vi "Destroy CIF Publisher.vi"(8 "error in (no error)":errorcluster, 11 "Publisher Reference":T1) -> (0 "error out":errorcluster)   [LabVIEW 2021, in "Iceoryx.lvlib"]
uses:
  Iceoryx.lvlib
  SubVIs/Convert Error Core.vi
  Refnum/Typedef/CIF Publisher Refnum.ctl
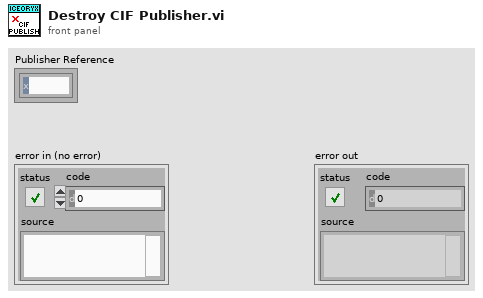
[diagram p1: front panel]
types:
  T1 = typedef "Iceoryx.lvlib/CIF Publisher Refnum.ctl" = refnum<k1>
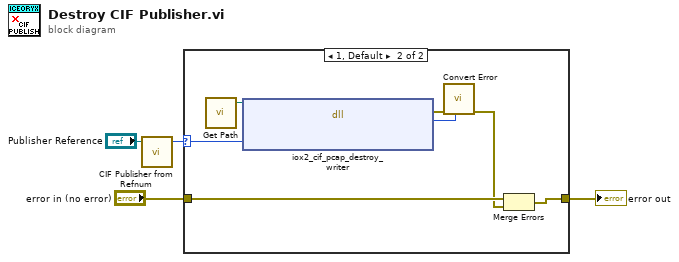
[diagram p0: block diagram]
diagram:
  n1 = call "CIF Publisher from Refnum.vi"("CIF Publisher Refnum"="Publisher Reference") -> ("CIF Publisher U64"=w1:u64)  [unwired: 4 in]
  n2 = case shown="1, Default" w1 {
    selector: w1 -> [_ w7]
    tunnel: "error in (no error)" -> [w5 w9]
    tunnel: [w5 w6] -> w2
    frame 0 {
    }
    frame 1, Default {
      n3 = call "Get Path.vi"() -> ("libiox2_cif path"=w12:path)  [unwired: 4 in]
      n4 = dll-call lib="D:/dev/iceoryx2_lvwrapper/dist/iox2_cif.dll" fn="iox2_cif_pcap_destroy_writer"(path in=w12, "writer"=w7) -> (error out=w11:errorcluster, "return type"=w10:i32)  [unwired: 3 in, 1 out]
      n5 = call "Convert Error.vi"("return type"=w10, "error in (no error)"=w11) -> ("error out"=w8:errorcluster)  [unwired: 9 in]
      n6 = Merge Errors(w9, w8) -> (w6:errorcluster)
    }
  }
  "error out" <- w2
